vi "Initialize and Finalize.vi"(8 "error in (no error)":errorcluster) -> (0 "error out":errorcluster)   [LabVIEW 2020]
uses:
  G-Embedded-Python-Interpreter-Toolkit/Merge Call Library Errors.vi
  <vilib>/addons/_JKI Toolkits/Caraya/classes/Assert/Assert Not Error.vi
  <vilib>/addons/_JKI Toolkits/Caraya/classes/Assert/Assert True.vi
  <vilib>/addons/_JKI Toolkits/Caraya/classes/Assert/Assert False.vi
  G-Embedded-Python-Interpreter-Toolkit/G-Embedded-Python-Interpreter-Toolkit.lvlib
  <vilib>/addons/_JKI Toolkits/Caraya/classes/Assert/Assert.lvclass
  <vilib>/addons/_JKI Toolkits/Caraya/classes/Test/Test.lvclass
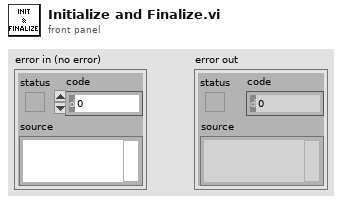
[diagram p1: front panel]
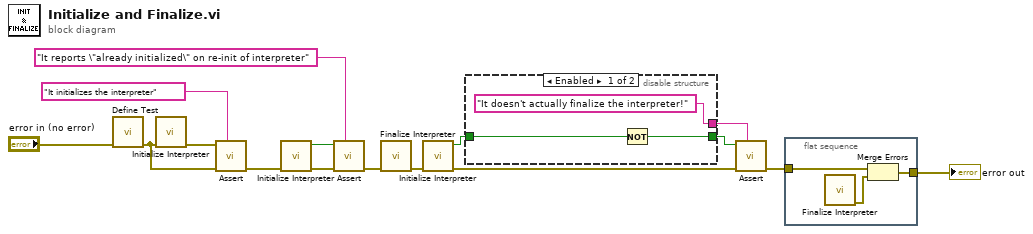
[diagram p0: block diagram]
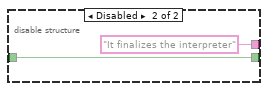
[diagram p2: hidden frame]
diagram:
  n1 = call <vilib>:"Define Test.vi"("error in (no error)"="error in (no error)") -> ("error out"=w15:errorcluster)  [unwired: 10 in]
  n2 = call "Initialize Interpreter.vi"("error in (no error)"=w15) -> ("error out"=w16:errorcluster)  [unwired: 9 in, 1 out]
  n3 = call-poly <vilib>:"Assert.vi"("Label"="It initializes the interpreter", "error in (no error)"=w15, "Not Error?"=w16) -> ("error out"=w13:errorcluster)  [unwired: 8 in]
  n4 = call "Initialize Interpreter.vi"("error in (no error)"=w13) -> ("error out"=w12:errorcluster, "Already Initialized"=w11:bool)  [unwired: 9 in]
  n5 = call-poly <vilib>:"Assert.vi"("Label"="It reports \"already initialized\" on re-init of interpreter", "error in (no error)"=w12, "True?"=w11) -> ("error out"=w9:errorcluster)  [unwired: 8 in]
  n6 = call "Finalize Interpreter.vi"("error in (no error)"=w9) -> ("error out"=w7:errorcluster)  [unwired: 10 in]
  n7 = call "Initialize Interpreter.vi"("error in (no error)"=w7) -> ("error out"=w6:errorcluster, "Already Initialized"=w2:bool)  [unwired: 9 in]
  n8 = disable-structure "Diagram Disable Structure" shown="Enabled" {
    disable-tunnel: [w17 w21] -> w3
    disable-tunnel: w2 -> [w18 w21]
    disable-tunnel: ["It doesn't actually finalize the interpreter!" ("Label") "It finalizes the interpreter" ("Label")] -> w1
    frame Enabled {
      n9 = Not(x=w18) -> (.not. x?=w17:bool)
    }
    frame Disabled {
    }
  }
  n10 = call-poly <vilib>:"Assert.vi"("Label"=w1, "error in (no error)"=w6, "False?"=w3) -> ("error out"=w4:errorcluster)  [unwired: 8 in]
  n11 = flat-sequence {
    tunnel: [w22] -> w5
    tunnel: w4 -> [w24]
    frame #0 {
      n12 = call "Finalize Interpreter.vi"() -> ("error out"=w23:errorcluster)  [unwired: 11 in]
      n13 = Merge Errors(w24, w23) -> (w22:errorcluster)
    }
  }
  "error out" <- w5
